vi "Create CIF Publisher.vi"(8 "error in (no error)":errorcluster, 10 "Universal":bool, 11 "CIF Pcap Publisher Configuration":T2) -> (0 "error out":errorcluster, 3 "CIF Publisher Refnum":T1 {"refnum" format="%.0x"})   [LabVIEW 2021, in "Iceoryx.lvlib"]
doc: "Create an iceoryx CIF pcap publisher. This can create up to two publisher queues, one with best effort that will overflow if the subscribers don't keep up, and one with backpressure which will block readers. If the numbr of subscribers for either is set to 0 it will not create that queue. \n\nMemory allocation is based on the max bytes, and number of subscribers. \nBest effort memory is (max bytes + 48) * (queue depth + number of subscribers + 1)\nBackpressure memory is (max bytes +48) * (queue depth +1) \n\nPublisher configuration:\n<B>Name:</B> Shared between multiple queue streams from the same source\n<B>Topic:</B> Unique name for this queue stream under the source name. Name/topic must be unique in the system\n<B>Link Type:</B> pcap Link Type used for subscriber type checks\n<B>Descriptor:</B> stored and can be read to help with parsing\n<B>Max Bytes, determines the maximum size of the pcap data elements \n<B>Best Effort Subscribers:</B> The number of best effort subscribers for the queue. More subscribers will allocate more memory. \n<B>Backpressure Subscribers:</B> The number of backpressure subscribers for the queue. Normally this is 0 or 1.\n<B>Best Effort Queue Depth:</B> how many elements deep is the queue\n<B>Backpressure Queue Depth:</B> how many elements deep is the queue\n\n<B>Universal:</B> Sets the subscriber to skip type check"
uses:
  Iceoryx.lvlib
  typedef/CIF Pcap Publisher Configuration.ctl
  Refnum/Typedef/CIF Publisher Refnum.ctl
  typedef/Errors.ctl
  SubVIs/Add Error Core.vi
  SubVIs/Convert Error Core.vi
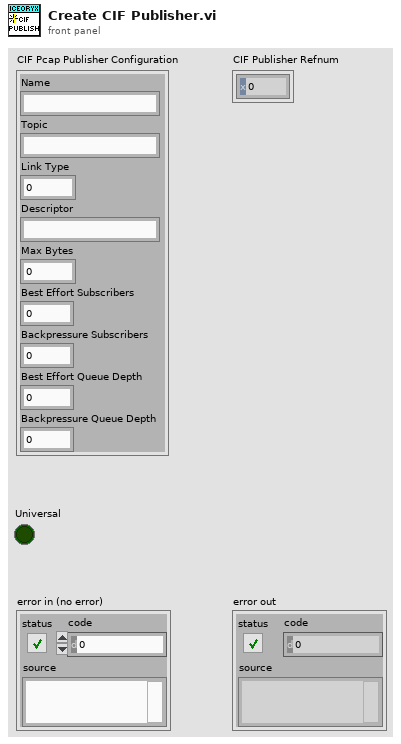
[diagram p1: front panel]
types:
  T1 = typedef "Iceoryx.lvlib/CIF Publisher Refnum.ctl" = cluster{"refnum":u64, "CIF Pub":enum8{"cifpub"}}
  T2 = typedef "Iceoryx.lvlib/CIF Pcap Publisher Configuration.ctl" = cluster{"Name":string, "Topic":string, "Link Type":u32, "Descriptor":string, "Max Bytes":u32, "Best Effort Subscribers":u32, "Backpressure Subscribers":u32, "Best Effort Queue Depth":u32, "Backpressure Queue Depth":u32}
  T3 = typedef "Iceoryx.lvlib/Errors.ctl" = enum16{"Unsupported Type", "Empty Name", "Cluster Name"}
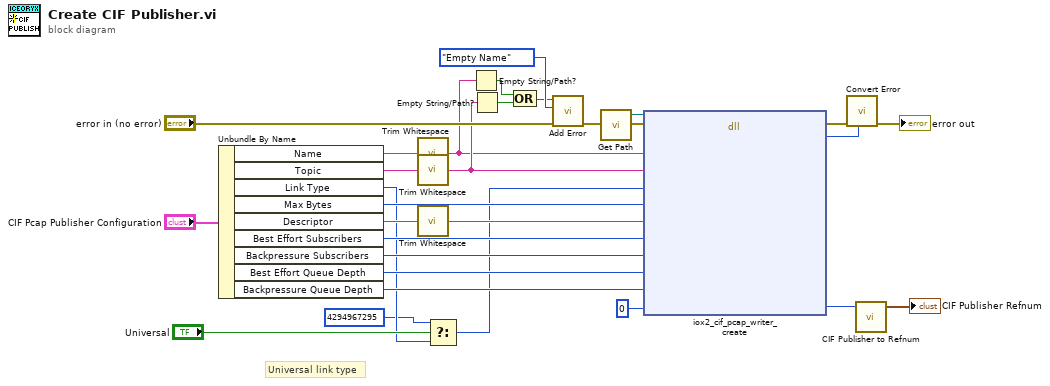
[diagram p0: block diagram]
diagram:
  # "Universal link type"
  n1 = Unbundle By Name("CIF Pcap Publisher Configuration") -> ("Name"=w21:string, "Topic"=w20:string, "Link Type"=w5:u32, "Max Bytes"=w12:u32, "Descriptor"=w14:string, "Best Effort Subscribers"=w11:u32, "Backpressure Subscribers"=w10:u32, "Best Effort Queue Depth"=w9:u32, "Backpressure Queue Depth"=w8:u32)
  n2 = call <vilib>:"Trim Whitespace.vi"("string"=w21) -> ("trimmed string"=w19:string)  [unwired: 1 in]
  n3 = call <vilib>:"Trim Whitespace.vi"("string"=w20) -> ("trimmed string"=w22:string)  [unwired: 1 in]
  n4 = call <vilib>:"Trim Whitespace.vi"("string"=w14) -> ("trimmed string"=w13:string)  [unwired: 1 in]
  n5 = Select(t=u32 4294967295, s="Universal", f=w5) -> (s? t:f=w3:u32)
  n6 = Empty String/Path?(string/path=w19) -> (empty?=w18:bool)
  n7 = Empty String/Path?(string/path=w22) -> (empty?=w17:bool)
  n8 = Compound Arithmetic op=OR(w18, w17) -> (w16:bool)
  n9 = call "Add Error.vi"("error in (no error)"="error in (no error)", "Error"=Errors."Empty Name", "Insert Error"=w16) -> ("error out"=w7:errorcluster)  [unwired: 8 in]
  n10 = call "Get Path.vi"() -> ("libiox2_cif path"=w26:path)  [unwired: 4 in]
  n11 = dll-call lib="D:/dev/iceoryx2_lvwrapper/dist/iox2_cif.dll" fn="iox2_cif_pcap_writer_create"(path in=w26, error in=w7, "name"=w19, "topic"=w22, "link_type"=w3, "max_pcap_bytes"=w12, "descriptor"=w13, "be_max_subscribers"=w11, "bp_max_subscribers"=w10, "be_subscriber_buffer"=w9, "bp_subscriber_buffer"=w8, "writer"=u64 0) -> (error out=w25:errorcluster, "return type"=w24:i32, "writer"=w2:u64)  [unwired: 10 in, 1 out]
  n12 = call "Convert Error.vi"("return type"=w24, "error in (no error)"=w25) -> ("error out"=→"error out":errorcluster)  [unwired: 9 in]
  n13 = call "CIF Publisher to Refnum.vi"("CIF Publisher U64"=w2) -> ("CIF Publisher Refnum"=→"CIF Publisher Refnum":T1)  [unwired: 4 in]
